vi "MaP traiter_donnees.vi"() -> ()   [LabVIEW 2020]
uses:
  LabVIEW-Python TCP Lib/LabVIEW-Python TCP Lib.lvlib
panel:
  in  "Server":string="\"D:\\Home\\eschaub\\Documents\\INFORMATIQUE\\LabVIEW-Python TCP\\Public repo\\Python\\lancer_serveur.py\""
  in  "port":u16=5000
  in  "Return data":T1
  in  "Sent data":T2={"fonction"="traiter_donnees", "parameters"={"nom"="convertir_majuscule", "valeur"=3.14, "configuration"={"coefficient"=1.5, "seuil"=0.8}}}
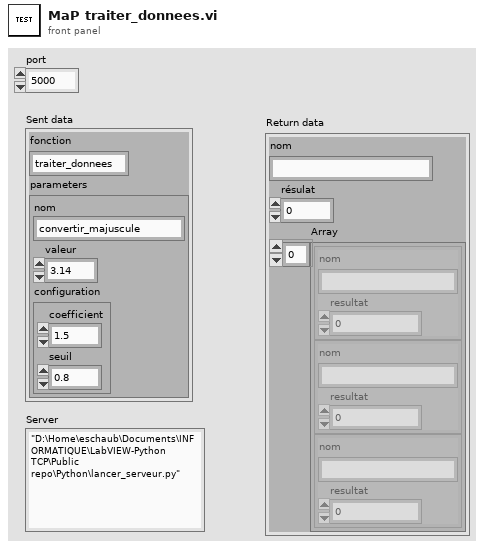
[diagram p1: front panel]
types:
  T1 = cluster{"nom":string, "résulat":dbl, "Array":cluster{"nom":string, "resultat":dbl}[]}
  T2 = cluster{"fonction":string, "parameters":cluster{"nom":string, "valeur":dbl, "configuration":cluster{"coefficient":dbl, "seuil":dbl}}}
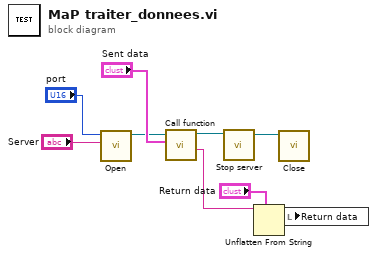
[diagram p0: block diagram]
diagram:
  n1 = call "Open.vi"("Lancer server.py"="Server", "port"="port") -> ("connection ID"=w2:refnum<k5>)  [unwired: 8 in, 1 out]
  n2 = call "Call function.vi"("variant in"="Sent data", "connection ID"=w2) -> ("data string out"=w6:string, "connection ID out"=w4:refnum<k5>)  [unwired: 6 in, 2 out]
  n3 = call "Stop server.vi"("connection ID"=w4) -> ("connection ID out"=w5:refnum<k5>)  [unwired: 8 in, 2 out]
  n4 = Unflatten From String(type="Return data", binary string=w6) -> (value=w8:T1)  [unwired: 3 in, 2 out]
  n5 = call "Close.vi"("connection ID"=w5) -> ()  [unwired: 9 in, 2 out]
  n6 = local write "Return data"(w8) -> ()
